vi "Begin.vi"(8 "error in":errorcluster) -> (0 "error out":errorcluster)   [LabVIEW 2017]
doc: "Called before other user functions, this VI can be used to open I/O refnums, load in file data, and do general program initialization. Notice that the <B>error out</B> terminal is simply used for data flow. Wiring it to other structures or subVIs ensures that this VI runs first."
uses:
  <vilib>/Rock Robotics/WPI/DriverStation/WPI_DriverStationRobotMode2.ctl
  <vilib>/Rock Robotics/WPI/Joystick/WPI_JoystickDeviceEnum.ctl
  Robot Global Data.vi
  <vilib>/Rock Robotics/Network Tables/NT Write String Array.vi
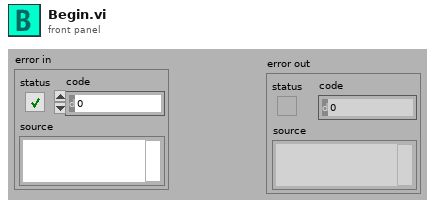
[diagram p1: front panel]
types:
  T1 = typedef "WPI_JoystickDeviceEnum.ctl" = enum16{"USB 0", "USB 1", "USB 2", "USB 3", "USB 4", "USB 5"}
  T2 = typedef "WPI_DriverStationRobotMode2.ctl" = enum16{"Autonomous Disabled", "Autonomous Enabled", "Teleop Disabled", "Teleop Enabled", "Disconnected", "Finish", "Test Disabled", "Test Enabled", "Emergency Stopped"}
  T3 = typedef "WPI_JoystickDevRef.ctl" = cluster{"Device":T1}
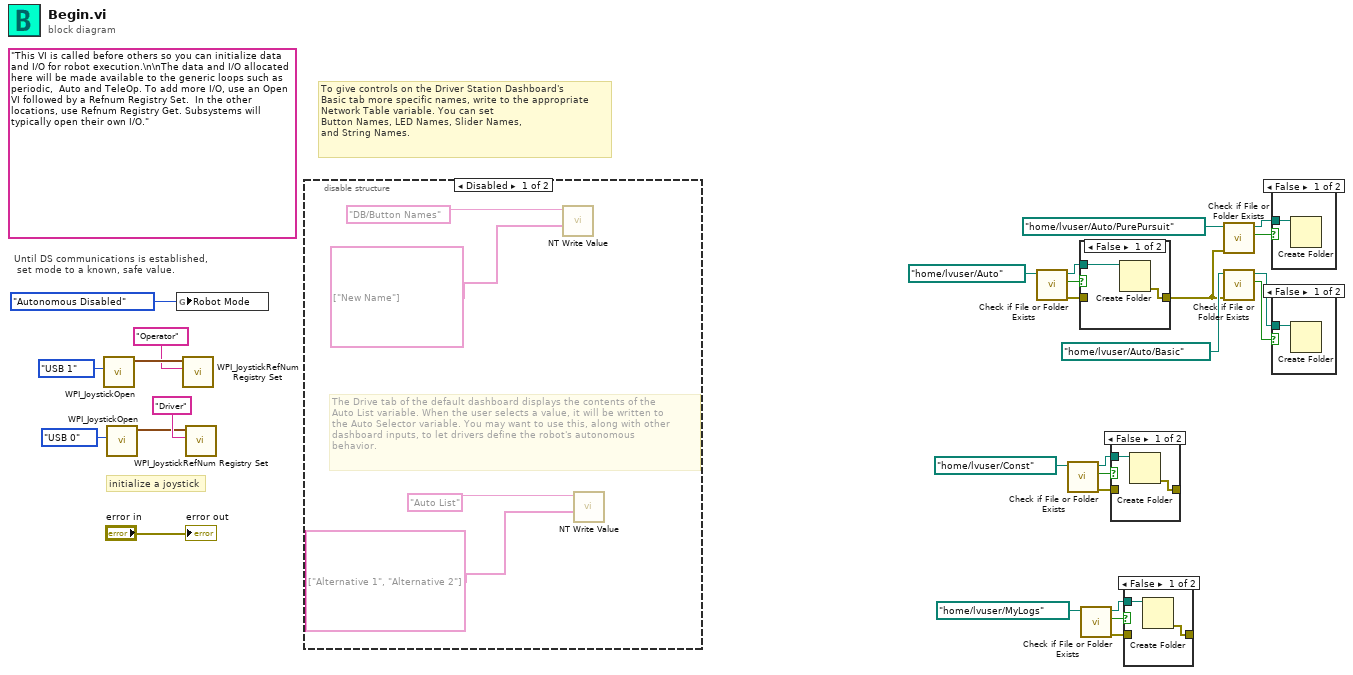
[diagram p0: block diagram]
diagram:
  (unwired) "This VI is called before others so you can initialize data and I/O for robot execution.\n\nThe data and I/O allocated here will be made available to the generic loops such as periodic,  Auto and TeleOp. To add more I/O, use an Open VI followed by a Refnum Registry Set.  In the other locations, use Refnum Registry Get. Subsystems will typically open their own I/O."
  # "To give controls on the Driver Station Dashboard's\nBasic tab more specific names, write to the appropriate\nNetwork Table variable. You can set\nButton Names, LED Names, Slider Names,\nand String Names."
  # "initialize a joystick"
  # "Until DS communications is established,\n set mode to a known, safe value."
  n1 = call <vilib>:"WPI_JoystickOpen.vi"("JoystickDevice"=WPI_JoystickDeviceEnum."USB 1") -> ("JoystickDevRef"=w2:T3)  [unwired: 10 in]
  n2 = call <vilib>:"WPI_JoystickOpen.vi"("JoystickDevice"=WPI_JoystickDeviceEnum."USB 0") -> ("JoystickDevRef"=w25:T3)  [unwired: 10 in]
  n3 = global write "Robot Global Data.vi" "Robot Mode"(WPI_DriverStationRobotMode2."Autonomous Disabled" ("Robot Mode")) -> ()
  n4 = call <vilib>:"WPI_JoystickRefNum Registry Set.vi"("refnum name"="Operator", "JoystickDevRef"=w2) -> ()  [unwired: 8 in, 2 out]
  n5 = call <vilib>:"WPI_JoystickRefNum Registry Set.vi"("refnum name"="Driver", "JoystickDevRef"=w25) -> ()  [unwired: 8 in, 2 out]
  n6 = disable-structure shown="Disabled" {
    frame Disabled {
      # "The Drive tab of the default dashboard displays the contents of the\nAuto List variable. When the user selects a value, it will be written to\nthe Auto Selector variable. You may want to use this, along with other\ndashboard inputs, to let drivers define the robot's autonomous\nbehavior."
      n7 = call-poly <vilib>:"NT Write Value.vi"("String Array"=string[] ["New Name"], "Name"="DB/Button Names") -> ()  [unwired: 9 in, 1 out]
      n8 = call-poly <vilib>:"NT Write Value.vi"("String Array"=string[] ["Alternative 1", "Alternative 2"], "Name"="Auto List") -> ()  [unwired: 9 in, 1 out]
    }
    frame Enabled {
    }
  }
  n9 = call <vilib>:"Check if File or Folder Exists.vi"("path"=path "/home/lvuser/Auto") -> ("error out"=w22:errorcluster, "file or folder exists?"=w21:bool, "dup path"=w20:path)  [unwired: 8 in]
  n10 = call <vilib>:"Check if File or Folder Exists.vi"("path"=path "/home/lvuser/Const") -> ("error out"=w8:errorcluster, "file or folder exists?"=w9:bool, "dup path"=w10:path)  [unwired: 8 in]
  n11 = case shown="False" w21 {
    tunnel: w20 -> [w33 _]
    tunnel: [w32 w34] -> w12
    tunnel: w22 -> [_ w34]
    frame False {
      n12 = Create Folder(path (use dialog)=w33) -> (error out=w32:errorcluster)  [unwired: 2 in, 2 out]
    }
    frame True {
    }
  }
  n13 = call <vilib>:"Check if File or Folder Exists.vi"("path"=path "/home/lvuser/MyLogs") -> ("error out"=w7:errorcluster, "file or folder exists?"=w6:bool, "dup path"=w5:path)  [unwired: 8 in]
  n14 = case shown="False" w9 {
    tunnel: w10 -> [w36 _]
    tunnel: [w35 w37] -> _
    tunnel: w8 -> [_ w37]
    frame False {
      n15 = Create Folder(path (use dialog)=w36) -> (error out=w35:errorcluster)  [unwired: 2 in, 2 out]
    }
    frame True {
    }
  }
  n16 = case shown="False" w6 {
    tunnel: w5 -> [w39 _]
    tunnel: [w38 w40] -> _
    tunnel: w7 -> [_ w40]
    frame False {
      n17 = Create Folder(path (use dialog)=w39) -> (error out=w38:errorcluster)  [unwired: 2 in, 2 out]
    }
    frame True {
    }
  }
  n18 = call <vilib>:"Check if File or Folder Exists.vi"("error in (no error)"=w12, "path"=path "/home/lvuser/Auto/PurePursuit") -> ("file or folder exists?"=w18:bool, "dup path"=w17:path)  [unwired: 7 in, 1 out]
  n19 = call <vilib>:"Check if File or Folder Exists.vi"("error in (no error)"=w12, "path"=path "/home/lvuser/Auto/Basic") -> ("file or folder exists?"=w14:bool, "dup path"=w15:path)  [unwired: 7 in, 1 out]
  n20 = case shown="False" w18 {
    tunnel: w17 -> [w41 _]
    frame False {
      n21 = Create Folder(path (use dialog)=w41) -> ()  [unwired: 2 in, 3 out]
    }
    frame True {
    }
  }
  n22 = case shown="False" w14 {
    tunnel: w15 -> [w42 _]
    frame False {
      n23 = Create Folder(path (use dialog)=w42) -> ()  [unwired: 2 in, 3 out]
    }
    frame True {
    }
  }
  "error out" <- "error in"
